vi "Base sp cluster selection for database and baseprofile.vi"(8 "error in":errorcluster) -> (0 "error out":errorcluster, 2 "element":string, 3 "Base All Composition":T1(array[cluster]))   [LabVIEW 2018]
panel:
  in  "Mode":bool
  in  "END":bool
  out "stripped path":path
  in  "selection":i32
  out "filenames":string[](array[string])
  out "Recipe#":i32
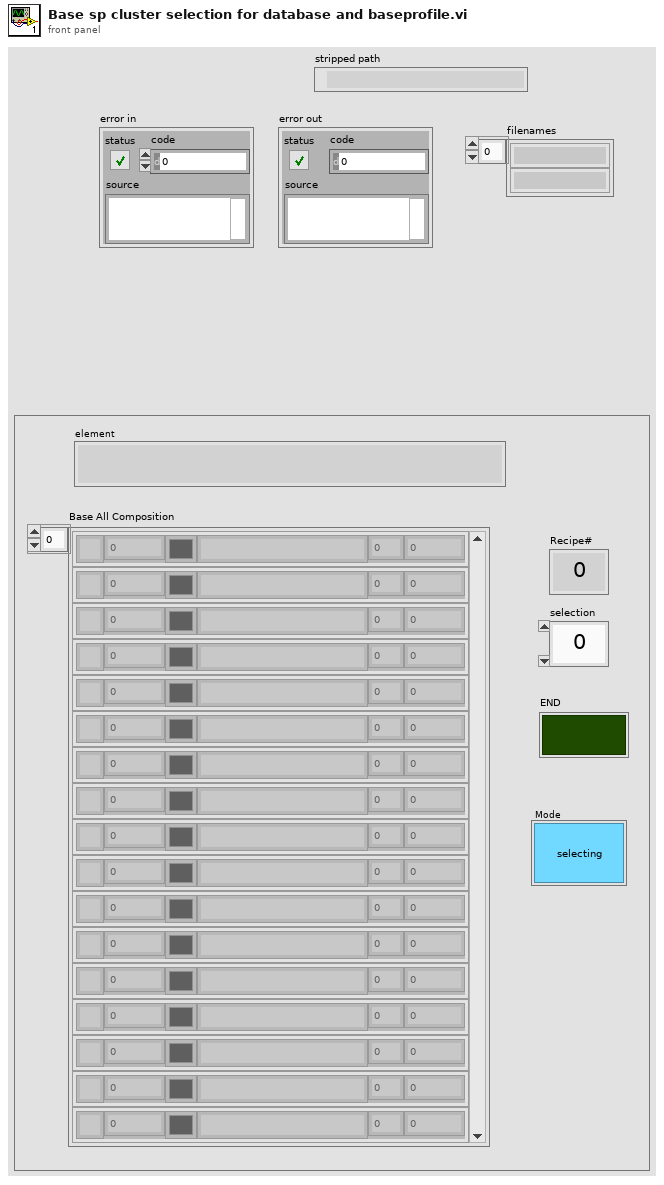
[diagram p1: front panel]
types:
  T1 = cluster{"Name":string, "Value":dbl, "Color":u32, "Name 2":string, "Value 2":dbl, "Value 3":dbl}[]
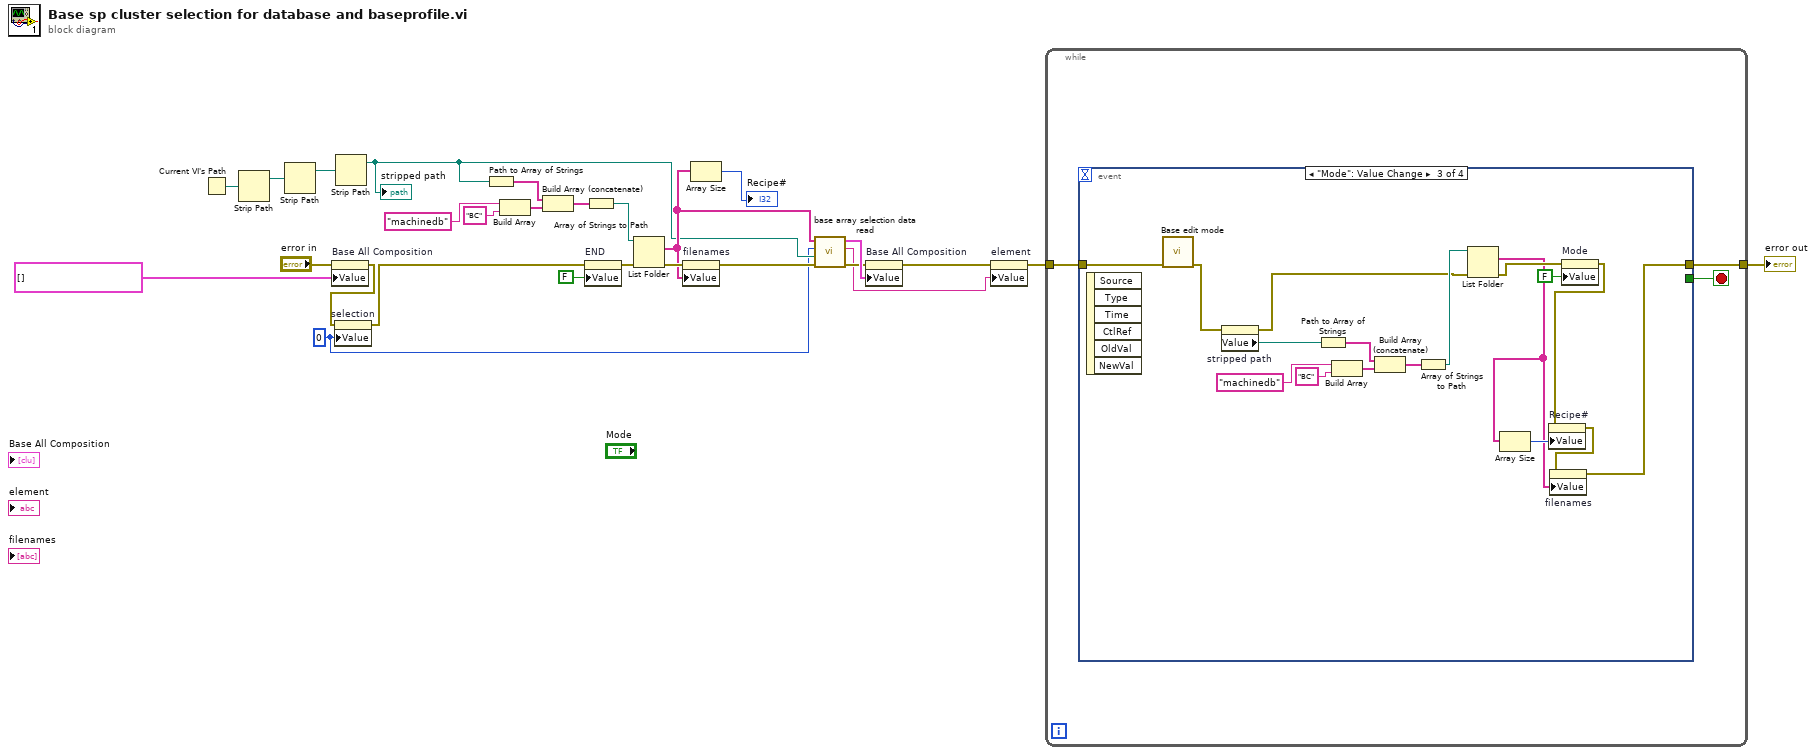
[diagram p0: block diagram]
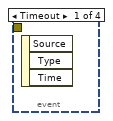
[diagram p2: hidden frame]
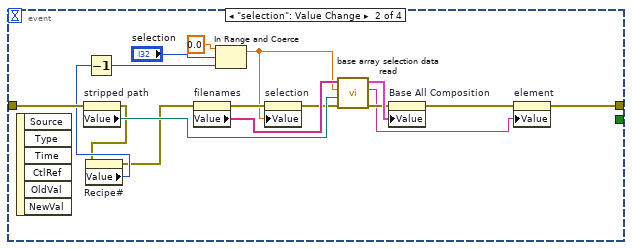
[diagram p3: hidden frame]
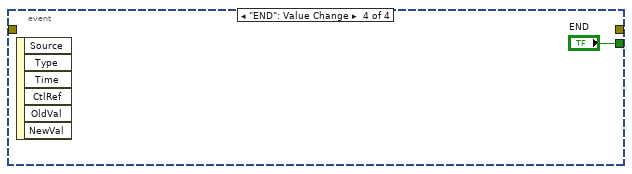
[diagram p4: hidden frame]
diagram:
  w1 = 0 ("selection")
  n1 = Current VI's Path() -> (path=w27:path)
  n2 = Strip Path(path=w27) -> (stripped path=w26:path)  [unwired: 1 out]
  n3 = Strip Path(path=w26) -> (stripped path=w25:path)  [unwired: 1 out]
  n4 = property on="Base All Composition" class="Arr (strict)"(error in="error in", "Value"=T1 [] ("Base All Composition 2")) -> (error out=w3:errorcluster)  [unwired: 1 in, 1 out]
  n5 = property on="selection" class="DigNum (strict)"(error in=w3, "Value"=w1) -> (error out=w2:errorcluster)  [unwired: 1 in, 1 out]
  n6 = Strip Path(path=w25) -> (stripped path=w10:path)  [unwired: 1 out]
  "stripped path" <- w10
  n7 = Path to Array of Strings(0:w10) -> (2:w21:string[])  [unwired: 1 out]
  n8 = Build Array("machinedb", "BC") -> (w22:string[])
  n9 = Build Array (concatenate)(w21, w22) -> (w20:string[])
  n10 = property on="END" class="Bool (strict)"(error in=w2, "Value"=FALSE ("END")) -> (error out=w15:errorcluster)  [unwired: 1 in, 1 out]
  n11 = Array of Strings to Path(0:w20) -> (2:w19:path)  [unwired: 1 in]
  n12 = List Folder(path=w19, error in=w15) -> (filenames=w11:string[], error out=w18:errorcluster)  [unwired: 2 in, 2 out]
  n13 = property on="filenames" class="Arr (strict)"(error in=w18, "Value"=w11) -> (error out=w12:errorcluster)  [unwired: 1 in, 1 out]
  n14 = Array Size(array=w11) -> (size(s)=→"Recipe#":i32)
  n15 = call "base array selection data read.vi"("error in"=w12, "stripped path"=w10, "selection"=w1, "filenames"=w11) -> ("error out"=w8:errorcluster, "element"=w7:string, "Base All Composition"=w9:T1)  [unwired: 5 in]
  n16 = property on="Base All Composition" class="Arr (strict)"(error in=w8, "Value"=w9) -> (error out=w6:errorcluster)  [unwired: 1 in, 1 out]
  n17 = property on="element" class="Str"(error in=w6, "Value"=w7) -> (error out=w5:errorcluster)  [unwired: 1 in, 1 out]
  n18 = while {
    tunnel: w5 -> [w30]
    tunnel: [w29] -> w17
    stop <- w28 stop-if-true
    n19 = event shown="[2] \"Mode\": Value Change" {
      selector: _ -> [_ _ _ _]
      dyn-events: _ -> [_ _ _ _]
      timeout: _ -> [_ _ _ _]
      tunnel: w30 -> [_ w47 w64 _]
      tunnel: [_ w40 w49 _] -> w29
      tunnel: [_ _ _ "END"] -> w28
      event Timeout {
        n20 = event-data() -> ()  [unwired: 1 in, 3 out]
      }
      event "selection": Value Change {
        n21 = event-data() -> ()  [unwired: 1 in, 6 out]
        n22 = property on="stripped path" class="Path"(error in=w47) -> (error out=w32:errorcluster, "Value"=w45:path)  [unwired: 1 in, 1 out]
        n23 = property on="Recipe#" class="DigNum (strict)"(error in=w32) -> (error out=w31:errorcluster, "Value"=w33:i32)  [unwired: 1 in, 1 out]
        n24 = Decrement(x=w33) -> (x-1=w34:i32)
        n25 = property on="filenames" class="Arr (strict)"(error in=w31) -> (error out=w37:errorcluster, "Value"=w46:string[])  [unwired: 1 in, 1 out]
        n26 = In Range and Coerce(upper limit=0.0, x="selection", lower limit=w34) -> (coerced(x)=w35:dbl)  [unwired: 1 out]
        n27 = property on="selection" class="DigNum (strict)"(error in=w37, "Value"=w35) -> (error out=w36:errorcluster)  [unwired: 1 in, 1 out]
        n28 = call "base array selection data read.vi"("error in"=w36, "stripped path"=w45, "selection"=w35, "filenames"=w46) -> ("error out"=w43:errorcluster, "element"=w42:string, "Base All Composition"=w44:T1)  [unwired: 5 in]
        n29 = property on="Base All Composition" class="Arr (strict)"(error in=w43, "Value"=w44) -> (error out=w41:errorcluster)  [unwired: 1 in, 1 out]
        n30 = property on="element" class="Str"(error in=w41, "Value"=w42) -> (error out=w40:errorcluster)  [unwired: 1 in, 1 out]
      }
      event "Mode": Value Change {
        n31 = event-data() -> ()  [unwired: 1 in, 6 out]
        n32 = call "Base edit mode.vi"("error in"=w64) -> ("error out"=w55:errorcluster)  [unwired: 9 in, 1 out]
        n33 = property on="stripped path" class="Path"(error in=w55) -> (error out=w54:errorcluster, "Value"=w57:path)  [unwired: 1 in, 1 out]
        n34 = Path to Array of Strings(0:w57) -> (2:w59:string[])  [unwired: 1 out]
        n35 = Build Array("machinedb", "BC") -> (w60:string[])
        n36 = Build Array (concatenate)(w59, w60) -> (w58:string[])
        n37 = Array of Strings to Path(0:w58) -> (2:w56:path)  [unwired: 1 in]
        n38 = List Folder(path=w56, error in=w54) -> (filenames=w48:string[], error out=w52:errorcluster)  [unwired: 2 in, 2 out]
        n39 = Array Size(array=w48) -> (size(s)=w53:i32)
        n40 = property on="Mode" class="Bool (strict)"(error in=w52, "Value"=FALSE ("Mode")) -> (error out=w51:errorcluster)  [unwired: 1 in, 1 out]
        n41 = property on="Recipe#" class="DigNum (strict)"(error in=w51, "Value"=w53) -> (error out=w50:errorcluster)  [unwired: 1 in, 1 out]
        n42 = property on="filenames" class="Arr (strict)"(error in=w50, "Value"=w48) -> (error out=w49:errorcluster)  [unwired: 1 in, 1 out]
      }
      event "END": Value Change {
        n43 = event-data() -> ()  [unwired: 1 in, 6 out]
      }
    }
  }
  "error out" <- w17
